vi "Read.vi"(8 "error in (no error)":errorcluster, 11 "DAQNavi_AI in":refnum<class "DAQNavi_AI.lvclass">) -> (0 "error out":errorcluster, 2 "Data Out":dbl format="%0.2f", 3 "DAQNavi_AI out":refnum<class "DAQNavi_AI.lvclass">)   [LabVIEW 2021, in "DAQNavi_AI.lvclass"]
uses:
  DAQNavi_AI.lvclass
  DAQNavi_AI.lvclass/DAQNavi_AI.ctl
  <userlib>/DAQNavi Polymorphic VI/read/DAQNavi Read (Analog DBL 1Chan 1Samp).vi
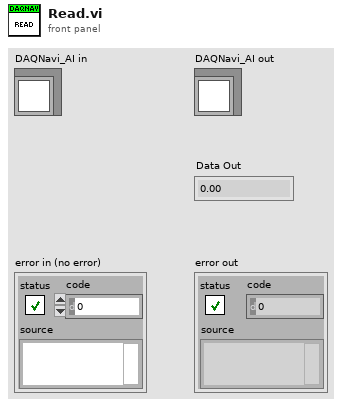
[diagram p1: front panel]
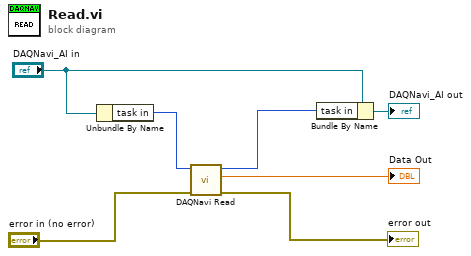
[diagram p0: block diagram]
diagram:
  n1 = Unbundle By Name("DAQNavi_AI in") -> ("task in"=w7:i32)
  n2 = call-poly <userlib>:"DAQNavi Read.vi"("error in (no error)"="error in (no error)", "task in"=w7) -> ("error out"=→"error out":errorcluster, "data"=→"Data Out":dbl, "task out"=w3:i32)  [unwired: 7 in]
  n3 = Bundle By Name(cluster="DAQNavi_AI in", "task in"=w3) -> (→"DAQNavi_AI out":refnum<class "DAQNavi_AI.lvclass">)
